vi "RDC-Lin-get_Dak35_Probe_info.vi"(7 "Enable bruteforce offset":bool) -> (2 "C0":dbl, 3 "Tau":dbl format="%#_6e")   [LabVIEW 2020, in "RDC-Reflection_Data_Computation.lvlib"]
doc: "Returns C0 and Tau of the DAK 3.5 probe, computed with RDC-Lin-Find_probe_char from open and short readings stored in the VI. Enable bruteforce offset adds stored offsets to C0 and Tau."
uses:
  RDC-Reflection_Data_Computation.lvlib
  Reflector/RFH-common_data_format.ctl
  Reflector/RFH-Reflection_File_Handler.lvlib
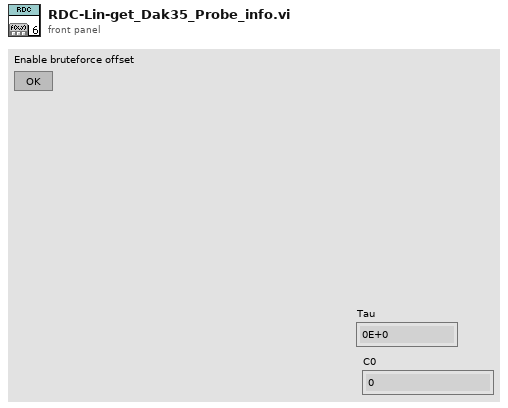
[diagram p1: front panel]
types:
  T1 = typedef "RFH-Reflection_File_Handler.lvlib/RFH-common_data_format.ctl" = cluster{"Frequency":dbl[], "Reflection'":dbl[], "Reflection''":dbl[], "Permativity'":dbl[], "Permativity''":dbl[], "Conductivity":dbl[], "Loss Tangent":dbl[], "Resistance":dbl[], "Reactance":dbl[]}
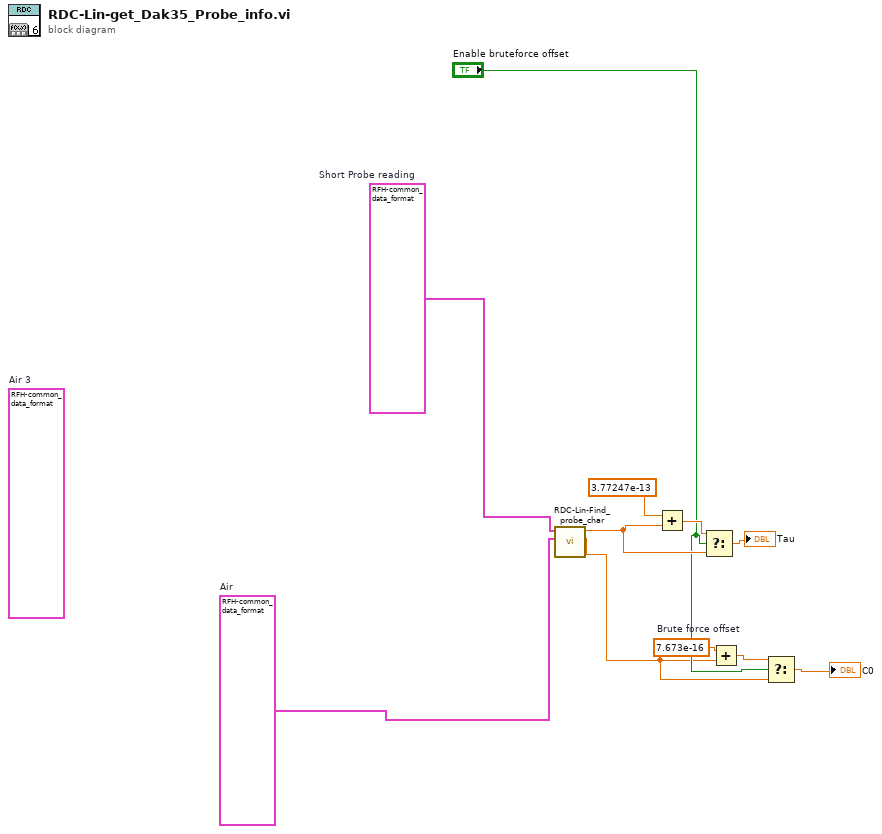
[diagram p0: block diagram]
diagram:
  w9 = 7.673e-16  # Brute force offset
  w10 = T1 {"Frequency"=array[2001 elements], "Reflection'"=array[2001 elements], "Reflection''"=array[2001 elements], "Permativity'"=array[2001 elements], "Permativity''"=array[2001 elements], "Conductivity"=array[2001 elements], "Loss Tangent"=array[2001 elements], "Resistance"=[], "Reactance"=[]}  # Air
  (unwired) T1 {"Frequency"=array[2001 elements], "Reflection'"=array[2001 elements], "Reflection''"=array[2001 elements], "Permativity'"=array[2001 elements], "Permativity''"=array[2001 elements], "Conductivity"=array[2001 elements], "Loss Tangent"=array[2001 elements], "Resistance"=[], "Reactance"=[]}  # Air 3
  w11 = T1 {"Frequency"=array[2001 elements], "Reflection'"=array[2001 elements], "Reflection''"=array[2001 elements], "Permativity'"=array[2001 elements], "Permativity''"=array[2001 elements], "Conductivity"=array[2001 elements], "Loss Tangent"=array[2001 elements], "Resistance"=[], "Reactance"=[]}  # Short Probe reading
  n1 = call "RDC-Lin-Find_probe_char.vi"("Open Probe reading"=w10, "Short Probe reading"=w11) -> ("C0"=w2:dbl, "Tau"=w7:dbl)  [unwired: 8 in]
  n2 = Add(x=3.77247e-13, y=w7) -> (x+y=w8:dbl)
  n3 = Select(t=w8, s="Enable bruteforce offset", f=w7) -> (s? t:f=→"Tau":dbl)
  n4 = Add(x=w9, y=w2) -> (x+y=w4:dbl)
  n5 = Select(t=w4, s="Enable bruteforce offset", f=w2) -> (s? t:f=→"C0":dbl)
